vi "Create Message VI (from Template).vi"(7 "replace string in template":string="package_templatemessage", 8 "error in (no error)":errorcluster, 9 "template VI name":string="Get package_templatemessage.vi", 10 "RPC Message Name":string, 11 "RPC Messages Folder (ProjectItem) in":refnum<vi>) -> (0 "error out":errorcluster, 1 "Created?":bool, 2 "Getter VI out":refnum<vi>, 3 "RPC Messages Folder (ProjectItem) out":refnum<vi>)   [LabVIEW 2019, in "gRPC Template Creation Utility.lvlib"]
uses:
  gRPC Template Creation Utility.lvlib
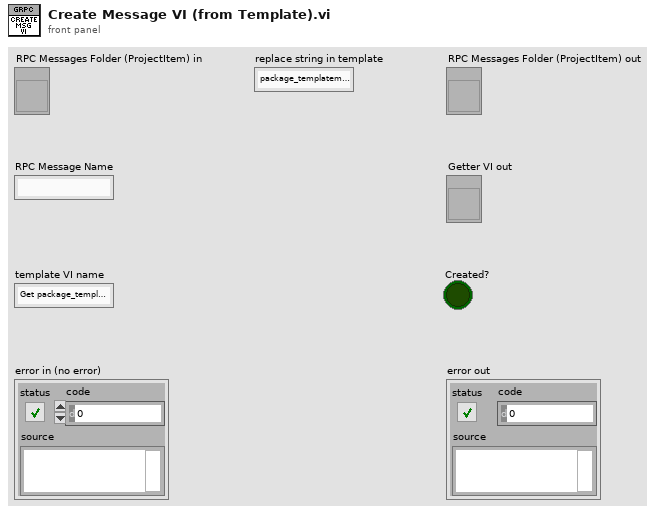
[diagram p1: front panel]
types:
  T1 = enum32{"invalid VI type", "Standard VI", "Control VI", "Global VI", "Polymorphic VI", "Configuration VI", "SubSystem", "Facade VI", "Method VI"}
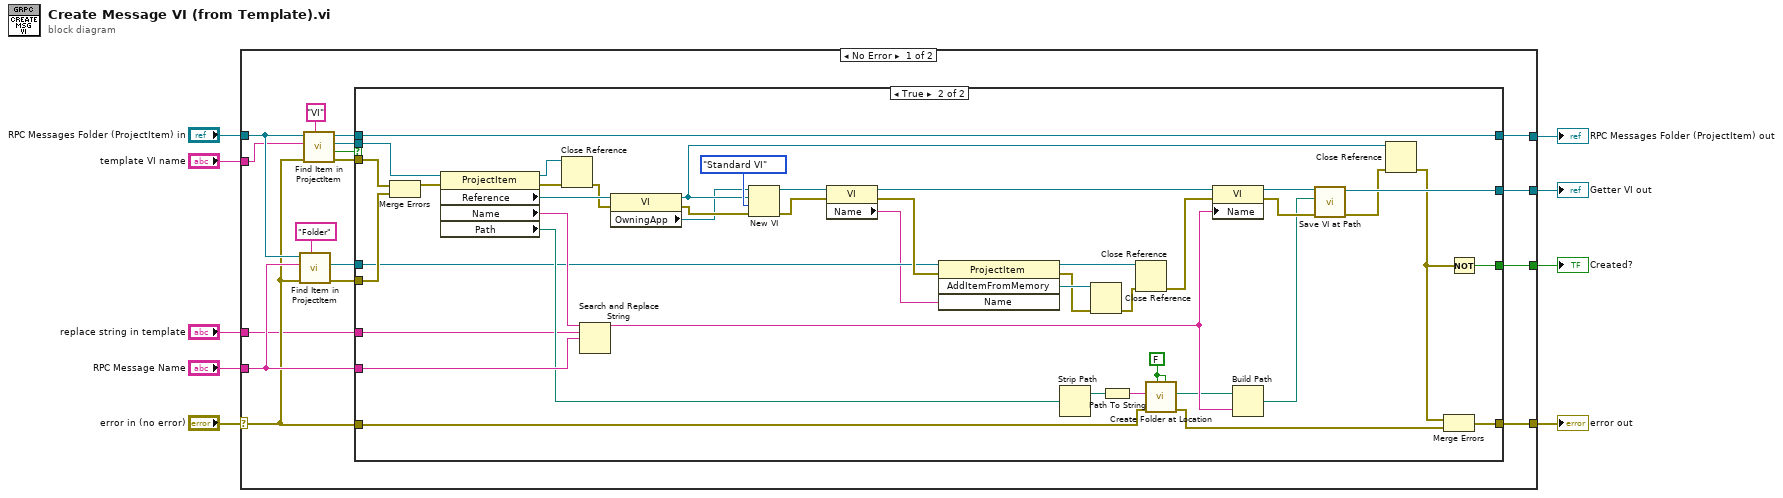
[diagram p0: block diagram]
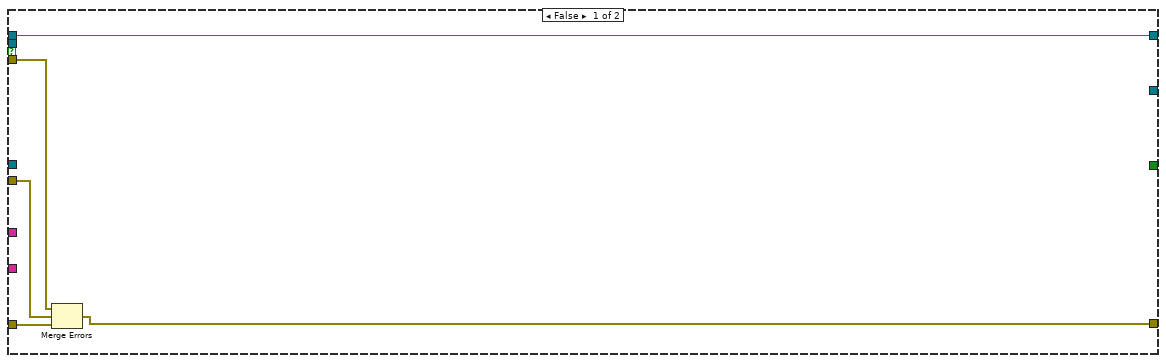
[diagram p2: hidden frame]
diagram:
  n1 = case shown="No Error" "error in (no error)" {
    selector: "error in (no error)" -> [w16 w75]
    tunnel: "RPC Message Name" -> [w26 _]
    tunnel: "RPC Messages Folder (ProjectItem) in" -> [w25 w76]
    tunnel: [w24 w75] -> w7
    tunnel: [w13 w76] -> w6
    tunnel: [w21 _] -> w5
    tunnel: [w12 _] -> w3
    tunnel: "template VI name" -> [w11 _]
    tunnel: "replace string in template" -> [w10 _]
    frame No Error {
      n2 = call "Find Item in ProjectItem.vi"("Item Type"="Folder", "error in (no error)"=w16, "Name"=w26, "ProjectItem in"=w25) -> ("error out"=w23:errorcluster, "Item Refnum out"=w20:refnum<vi>)  [unwired: 4 in, 2 out]
      n3 = call "Find Item in ProjectItem.vi"("Item Type"="VI", "error in (no error)"=w16, "Name"=w11, "ProjectItem in"=w25) -> ("error out"=w22:errorcluster, "Found ?"=w15:bool, "Item Refnum out"=w19:refnum<vi>, "ProjectItem out"=w14:refnum<vi>)  [unwired: 4 in]
      n4 = case shown="True" w15 {
        tunnel: w26 -> [_ w74]
        tunnel: [w29 w71] -> w24
        tunnel: w23 -> [w27 w69]
        tunnel: w22 -> [w28 w67]
        tunnel: [_ w65] -> w21
        tunnel: w20 -> [_ w54]
        tunnel: w19 -> [_ w49]
        tunnel: w16 -> [w30 w48]
        tunnel: w14 -> [w31 w47]
        tunnel: [w31 w47] -> w13
        tunnel: [_ w44] -> w12
        tunnel: w10 -> [_ w37]
        frame False {
          n5 = Merge Errors(w28, w27, w30) -> (w29:errorcluster)
        }
        frame True {
          w66 = FALSE ("Use Relative (F)")
          n6 = Merge Errors(w67, w69) -> (w68:errorcluster)
          n7 = property class="ProjectItem"(reference=w49, error in=w68) -> (reference out=w73:refnum<vi>, error out=w72:errorcluster, "Reference"=w36:refnum<vi>, "Name"=w57:string, "Path"=w56:path)
          n8 = Close Reference(reference=w73, error in (no error)=w72) -> (error out=w34:errorcluster)
          n9 = Search and Replace String(input string=w57, search string=w37, replace string=w74) -> (result string=w61:string)  [unwired: 5 in, 3 out]
          n10 = property class="VI"(reference=w36, error in=w34) -> (reference out=w35:refnum<vi>, error out=w33:errorcluster, "OwningApp"=w32:refnum<vi>)
          n11 = New VI(8:w33, 9:T1."Standard VI" ("vi type (standard vi)"), 10:w35, 11:w32) -> (0:w52:errorcluster, 3:w50:refnum<vi>)  [unwired: 3 out]
          n12 = property class="VI"(reference=w50, error in=w52) -> (reference out=w58:refnum<vi>, error out=w59:errorcluster, "Name"=w53:string)
          n13 = invoke class="ProjectItem" method="AddItemFromMemory"(reference=w54, error in=w59, "Name"=w53) -> (reference out=w46:refnum<vi>, error out=w42:errorcluster, "AddItemFromMemory"=w43:refnum<vi>)  [unwired: 1 in, 1 out]
          n14 = Strip Path(path=w56) -> (stripped path=w38:path)  [unwired: 1 out]
          n15 = Close Reference(reference=w43, error in (no error)=w42) -> (error out=w41:errorcluster)
          n16 = Path To String(path=w38) -> (string=w55:string)
          n17 = Close Reference(reference=w46, error in (no error)=w41) -> (error out=w45:errorcluster)
          n18 = call "Create Folder at Location.vi"("Override existing (F)"=w66, "Use Relative (F)"=w66, "Error In"=w48, "Path"=w55) -> ("Error Out"=w70:errorcluster, "Full path out"=w60:path)  [unwired: 5 in, 1 out]
          n19 = property class="VI"(reference=w58, error in=w45, "Name"=w61) -> (reference out=w62:refnum<vi>, error out=w64:errorcluster)
          n20 = Build Path(base path=w60, name or relative path=w61) -> (appended path=w63:path)
          n21 = call "Save VI at Path.vi"("error in (no error)"=w64, "Path"=w63, "VI in"=w62) -> ("error out"=w40:errorcluster, "VI out"=w65:refnum<vi>)  [unwired: 6 in, 1 out]
          n22 = Close Reference(reference=w35, error in (no error)=w40) -> (error out=w39:errorcluster)
          n23 = Merge Errors(w39, w70) -> (w71:errorcluster)
          n24 = Not(x=w39) -> (.not. x?=w44:bool)
        }
      }
    }
    frame Error {
    }
  }
  "error out" <- w7
  "RPC Messages Folder (ProjectItem) out" <- w6
  "Getter VI out" <- w5
  "Created?" <- w3
